vi "Configure.vi"(8 "error in (no error)":errorcluster, 11 "ImageHandler:DT-ImageHandler in":refnum<class "DT-ImageHandler.lvclass">) -> (0 "error out":errorcluster, 3 "ImageHandler:DT-ImageHandler out":refnum<class "DT-ImageHandler.lvclass">)   [LabVIEW 2022 SP3, in "ImageHandler.lvlib" / "DT-ImageHandler.lvclass"]
uses:
  DT-ImageHandler.lvclass
  DT-ImageHandler.lvclass/DT-ImageHandler.ctl
  xPanelWrapperLvLib/xPanelWrapper.lvlib
panel:
  out "nHeight out":u16
  out "nWidth out":u16
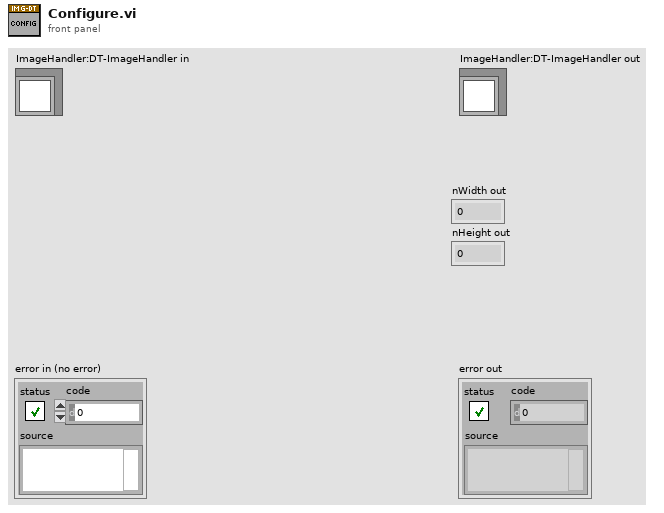
[diagram p1: front panel]
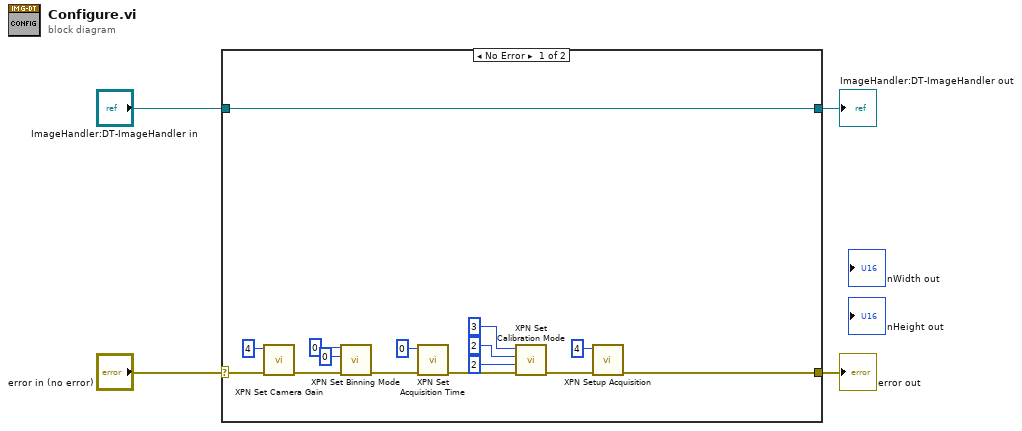
[diagram p0: block diagram]
diagram:
  n1 = case shown="No Error" "error in (no error)" {
    selector: "error in (no error)" -> [w18 w21]
    tunnel: [w13 w21] -> w3
    tunnel: [w19 w20] -> w1
    tunnel: "ImageHandler:DT-ImageHandler in" -> [w19 w20]
    frame No Error {
      n2 = call "XPN Set Camera Gain.vi"("error in (no error)"=w18, "gainMode"=4) -> ("error out"=w16:errorcluster)  [unwired: 8 in, 1 out]
      n3 = call "XPN Set Binning Mode.vi"("error in (no error)"=w16, "accumulated"=0, "binningMode"=0) -> ("error out"=w15:errorcluster)  [unwired: 7 in, 1 out]
      n4 = call "XPN Set Acquisition Time.vi"("error in (no error)"=w15, "timeMs"=0) -> ("error out"=w17:errorcluster)  [unwired: 8 in, 1 out]
      n5 = call "XPN Set Calibration Mode.vi"("error in (no error)"=w17, "defectMode"=2 ("offsetMode"), "gainMode"=2 ("offsetMode"), "offsetMode"=3) -> ("error out"=w14:errorcluster)  [unwired: 6 in, 1 out]
      n6 = call "XPN Setup Acquisition.vi"("error in (no error)"=w14, "ringBuffCount"=4) -> ("error out"=w13:errorcluster)  [unwired: 8 in, 1 out]
    }
    frame Error {
    }
  }
  "error out" <- w3
  "ImageHandler:DT-ImageHandler out" <- w1
